vi "Write Samples.vi"(8 "error in (no error)":errorcluster, 10 "Samples":refnum<class "Sample.lvclass">[](array[class]), 11 "Metric in":refnum<class "Metric.lvclass">) -> (0 "error out":errorcluster, 3 "Metric out":refnum<class "Metric.lvclass">)   [LabVIEW 2020]
uses:
  Metric.lvclass
  sample/Sample.lvclass
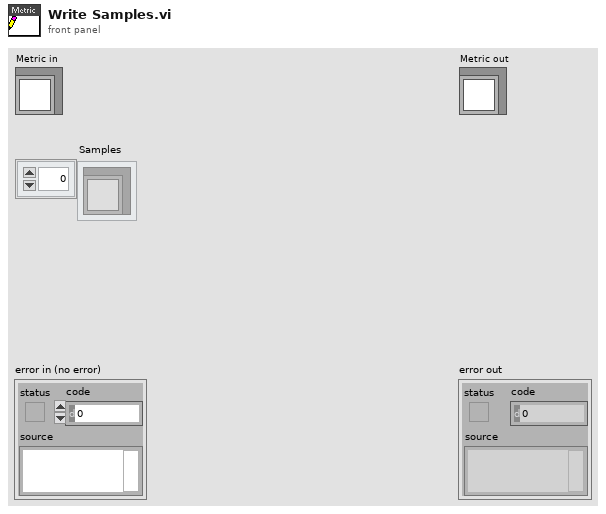
[diagram p1: front panel]
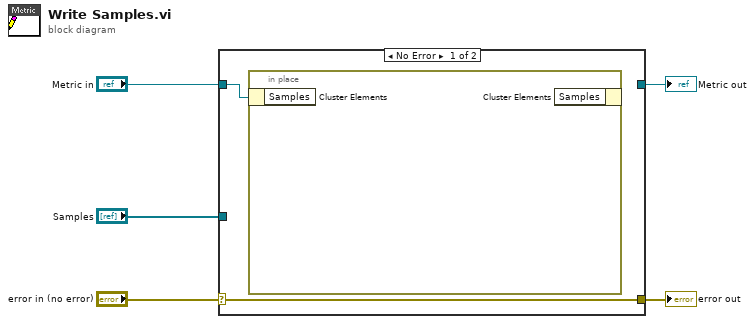
[diagram p0: block diagram]
diagram:
  n1 = case shown="No Error" "error in (no error)" {
    selector: "error in (no error)" -> [w7 w9]
    tunnel: [w7 w9] -> w4
    tunnel: [_ w10] -> w2
    tunnel: "Metric in" -> [w6 w10]
    tunnel: "Samples" -> [_ _]
    frame No Error {
      n2 = in-place {
        n3 = in-place-cluster #1(w6) -> ()  [unwired: 1 out]
        n4 = in-place-cluster #1() -> ("Samples"=w8)  [unwired: 1 out]
      }
    }
    frame Error {
    }
  }
  "error out" <- w4
  "Metric out" <- w2
